vi "VHist - coerce time to midnight.vi"(4 "time":dbl) -> (1 "midnight":dbl)   [LabVIEW 2021]
doc: "::: CalcExpress Toolkit :::\nCopyright (c) 2000-2026 Konstantin Shifershteyn. All rights reserved."
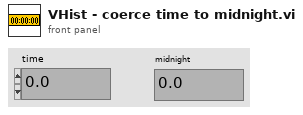
[diagram p1: front panel]
types:
  T1 = typedef "LVDateTimeRec.ctl" = cluster{"fractional second":dbl, "second":i32, "minute":i32, "hour":i32, "day of month":i32, "month":i32, "year":i32, "day of week":i32, "day of year":i32, "DST":i32}
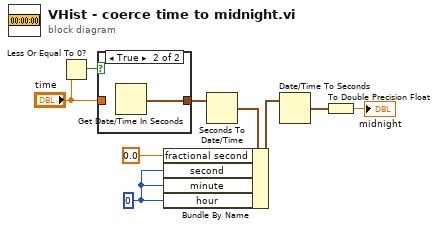
[diagram p0: block diagram]
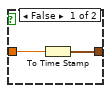
[diagram p2: hidden frame]
diagram:
  w8 = 0 ("hour")
  n1 = Less Or Equal To 0?(x="time") -> (x <= 0?=w5:bool)
  n2 = case shown="True" w5 {
    tunnel: [w11 w12] -> w6
    tunnel: "time" -> [w10 _]
    frame False {
      n3 = To Time Stamp(1:w10) -> (0:w11:timestamp)
    }
    frame True {
      n4 = Get Date/Time In Seconds() -> (seconds since 1Jan1904=w12:timestamp)
    }
  }
  n5 = Seconds To Date/Time(time stamp (now)=w6) -> (date time rec=w9:T1)  [unwired: 1 in]
  n6 = Bundle By Name(cluster=w9, "fractional second"=0.0, "second"=w8, "minute"=w8, "hour"=w8) -> (w3:T1)
  n7 = Date/Time To Seconds(2:w3) -> (0:w7:timestamp)  [unwired: 1 in]
  n8 = To Double Precision Float(number=w7) -> (double precision float=→"midnight":dbl)
